vi "Measurement Logic.vi"(6 "NI GUID":string, 8 "error in":errorcluster, 9 "measurement configuration":T2 {"Baudrate" format="%x"; "FD Baudrate" format="%x"}, 10 "measure call context in":refnum<class "Measure Call Context.lvclass">, 11 "Stop OOB Server UE":refnum<user-event>) -> (0 "error out":errorcluster, 1 "measurement results":T1, 2 "measure call context out":refnum<class "Measure Call Context.lvclass">)   [LabVIEW 2025, in "CAN-LIN Raw Bus Capture.lvclass"]
doc: "Contains the core logic for executing the measurement."
uses:
  CAN-LIN Raw Bus Capture.lvclass
  <vilib>/Plug-In SDKs/Measurements/Measure Call Context/Measure Call Context.lvclass
  Measurement Configuration.ctl
  CAN-LIN Raw Bus Capture UI/Toggle.ctl
  Measurement Results.ctl
  Logic Data.ctl
  State.ctl
  Create Frame Buffer.vi
  <vilib>/xnet/xnet.llb/XNET Read (Frame LIN).vi
  <vilib>/xnet/xnet.llb/XNET Read (State LIN Comm).vi
  <vilib>/xnet/xnet.llb/XNET Read (Frame CAN).vi
  <vilib>/xnet/xnet.llb/XNET Read (State CAN Comm).vi
  Enqueue Frame.vi
  Destroy Frame Buffer.vi
  CAN-LIN Raw Bus Capture.lvclass/CAN-LIN Raw Bus Capture.ctl
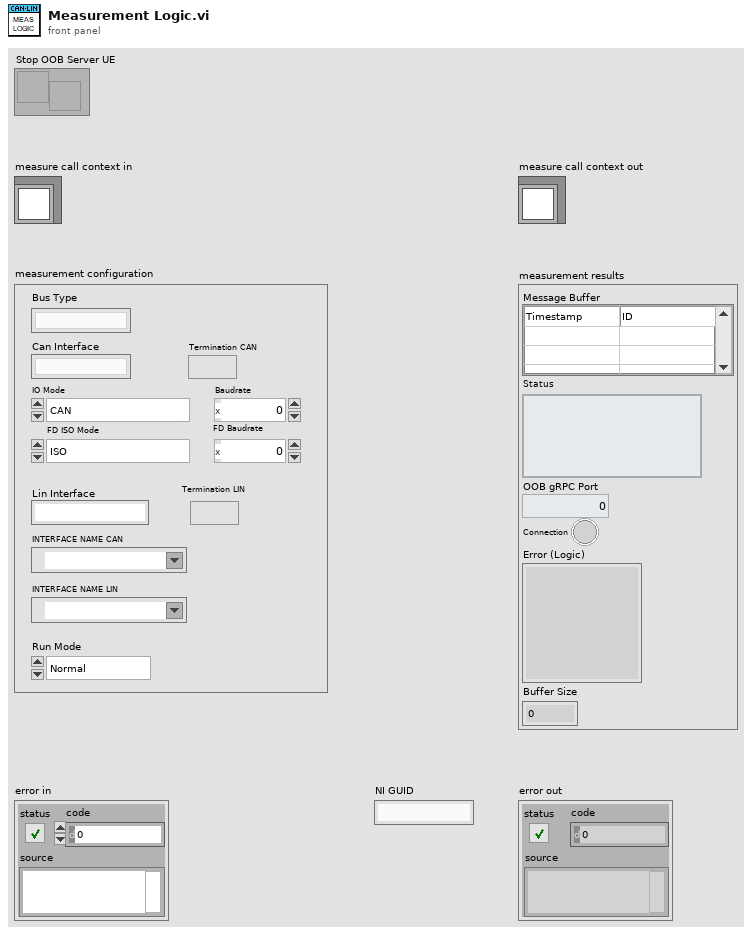
[diagram p1: front panel]
types:
  T1 = typedef "CAN-LIN Raw Bus Capture.lvclass/Measurement Results.ctl" = cluster{"Message Buffer":string[][], "Status":string, "OOB gRPC Port":i32, "Connection":bool, "Error (Logic)":string, "Buffer Size":i32}
  T2 = typedef "CAN-LIN Raw Bus Capture.lvclass/Measurement Configuration.ctl" = cluster{"Termination CAN":T3, "FD Baudrate":u32, "Baudrate":u32, "FD ISO Mode":enum32{"ISO", "Legacy ISO", "Non-ISO"}, "IO Mode":enum32{"CAN", "CAN FD", "CAN FD + BRS"}, "Termination LIN":T3, "Can Interface":string, "Lin Interface":string, "Bus Type":string, "INTERFACE NAME CAN":refnum<k21>, "INTERFACE NAME LIN":refnum<k21>, "Run Mode":enum32{"Normal", "Subordinate"}}
  T3 = typedef "Toggle.ctl" = bool
  T4 = typedef "CAN-LIN Raw Bus Capture.lvclass/Logic Data.ctl" = cluster{"State":T5, "Results":T1, "XNET Session":refnum<k21>}
  T5 = typedef "CAN-LIN Raw Bus Capture.lvclass/State.ctl" = enum16{"Init", "Execute", "Results", "Error", "Close"}
  T6 = typedef "XNET Frame LIN.ctl" = cluster{"timestamp":timestamp, "payload":u8[], "identifier":u32, "type":T7, "event ID":u8, "event slot?":bool, "echo?":bool}
  T7 = typedef "XNET Frame Type LIN.ctl" = u8
  T8 = typedef "XNET LIN Comm.ctl" = cluster{"fault code":i32, "fault?":bool, "communication state":T9, "last error":T10, "last error received":u8, "last error expected":u8, "last error identifier":u8, "sleep?":bool, "transceiver ready?":bool, "schedule index":u8}
  T9 = typedef "XNET LIN Comm State.ctl" = u8
  T10 = typedef "XNET LIN Last Err.ctl" = u8
  T11 = typedef "XNET Frame CAN.ctl" = cluster{"timestamp":timestamp, "payload":u8[], "identifier":u32, "type":T12, "extended?":bool, "echo?":bool}
  T12 = typedef "XNET Frame Type CAN.ctl" = u8
  T13 = typedef "XNET CAN Comm.ctl" = cluster{"fault code":i32, "fault?":bool, "communication state":T14, "last error":T15, "receive error counter":u8, "transmit error counter":u8, "transceiver error?":bool, "sleep?":bool}
  T14 = typedef "XNET CAN Comm State.ctl" = u8
  T15 = typedef "XNET CAN Last Err.ctl" = u8
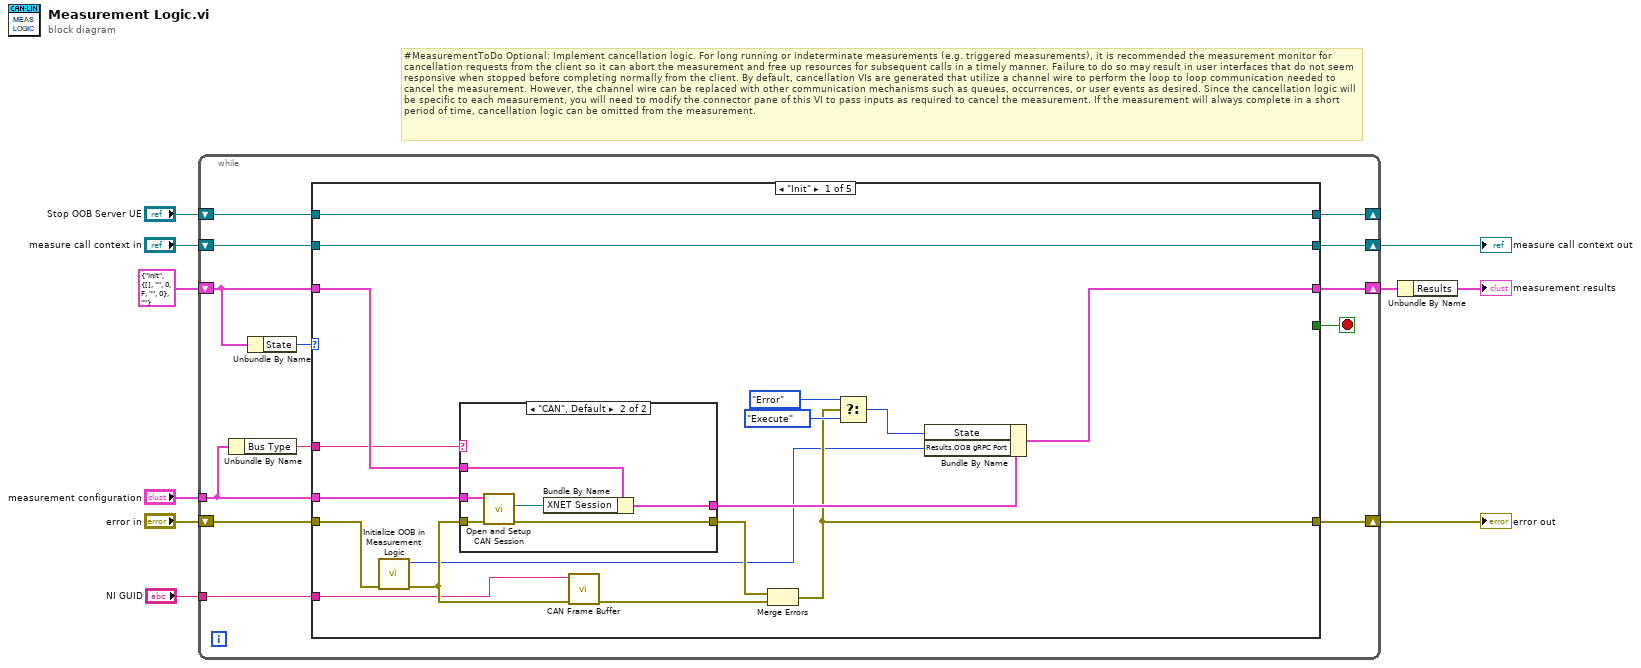
[diagram p0: block diagram]
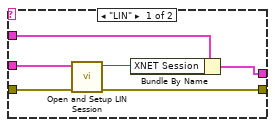
[diagram p2: hidden frame]
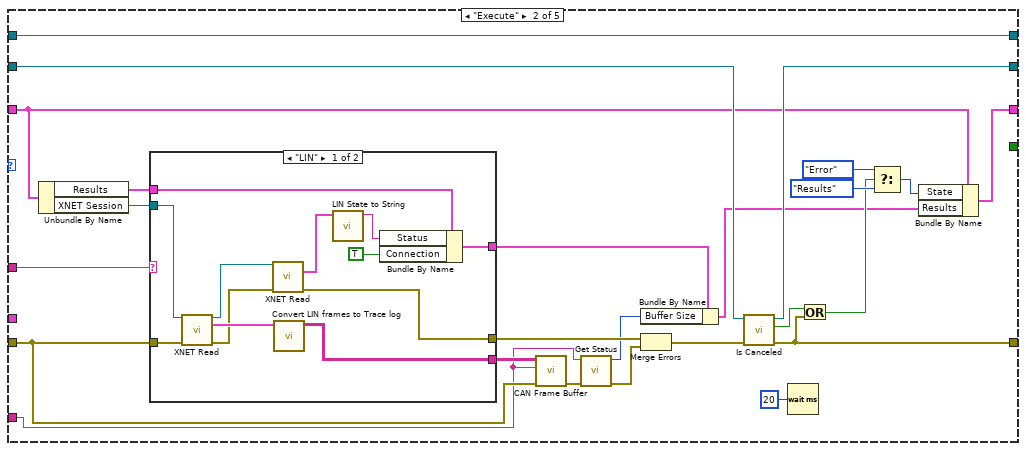
[diagram p3: hidden frame]
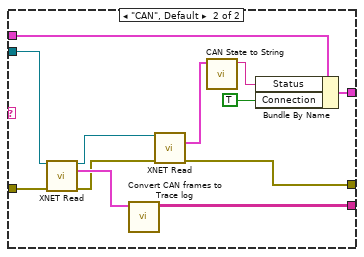
[diagram p4: hidden frame]
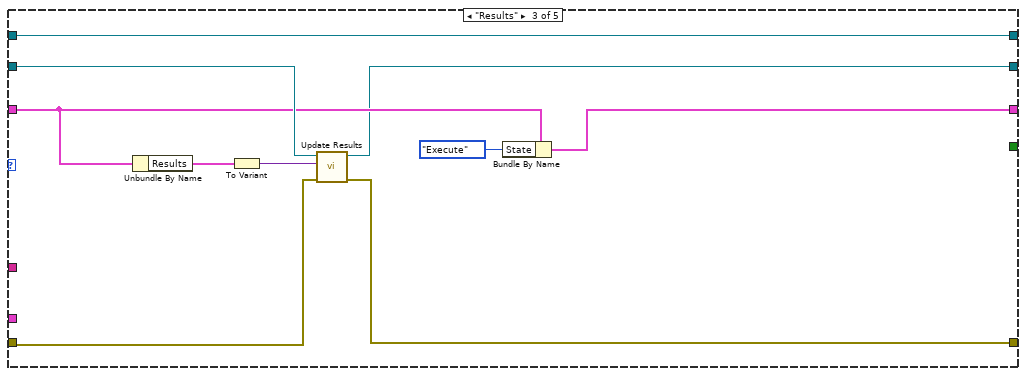
[diagram p5: hidden frame]
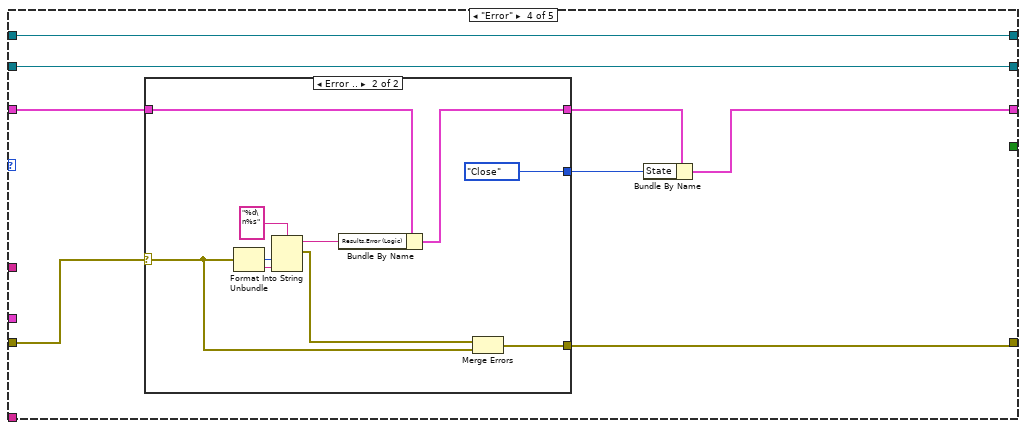
[diagram p6: hidden frame]
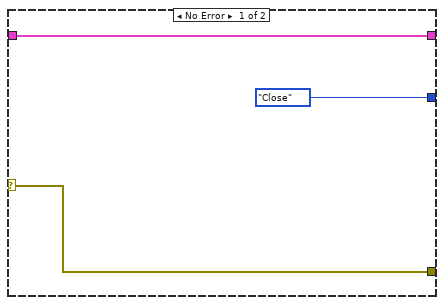
[diagram p7: hidden frame]
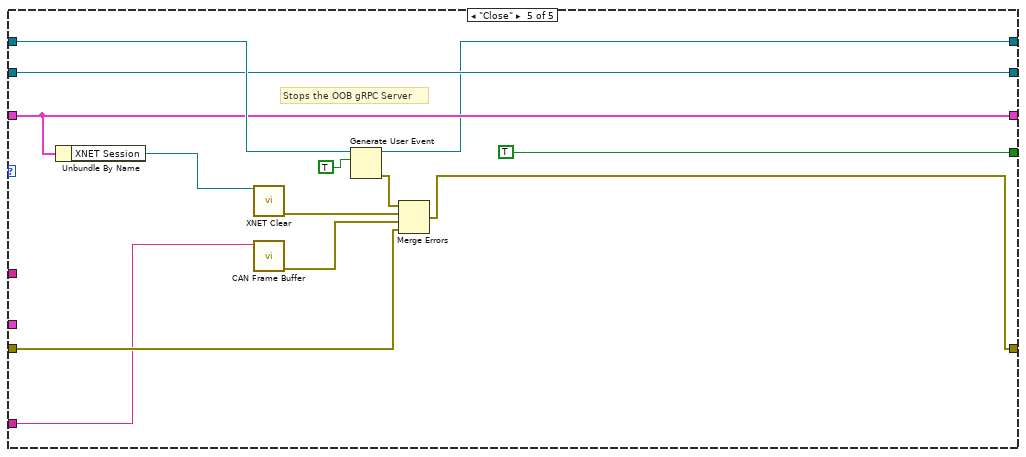
[diagram p8: hidden frame]
diagram:
  # "#MeasurementToDo Optional: Implement cancellation logic. For long running or indeterminate measurements (e.g. triggered measurements), it is recommended the measurement monitor for cancellation requests from the client so it can abort the measurement and free up resources for subsequent calls in a timely manner. Failure to do so may result in user interfaces that do not seem responsive when stopped before completing normally from the client. By default, cancellation VIs are generated that utilize a channel wire to perform the loop to loop communication needed to cancel the measurement. However, the channel wire can be replaced with other communication mechanisms such as queues, occurrences, or user events as desired. Since the cancellation logic will be specific to each measurement, you will need to modify the connector pane of this VI to pass inputs as required to cancel the measurement. If the measurement will always complete in a short period of time, cancellation logic can be omitted from the measurement."
  n1 = while {
    shift-right: [w19] -> w7
    shift-left: "error in" -> [w18]
    shift-right: [w20] -> w6
    shift-left: "measure call context in" -> [w23]
    shift-right: [w15] -> w3
    shift-left: T4 {"State"=enum."Init", "Results"={"Message Buffer"=[], "Status"="", "OOB gRPC Port"=0, "Connection"=FALSE, "Error (Logic)"="", "Buffer Size"=0}, "XNET Session"=""} ("Logic Data") -> [w16]
    tunnel: "measurement configuration" -> [w14]
    shift-right: [w12] -> _
    shift-left: "Stop OOB Server UE" -> [w22]
    tunnel: "NI GUID" -> [w11]
    stop <- w21 stop-if-true
    n2 = Unbundle By Name(w14) -> ("Bus Type"=w13:string)
    n3 = Unbundle By Name(w16) -> ("State"=w17:T5)
    n4 = case shown="\"Init\"" w17 {
      tunnel: w23 -> [w33 w73 w111 w113 w143]
      tunnel: w22 -> [w28 w57 w104 w112 w145]
      tunnel: [_ _ _ _ TRUE] -> w21
      tunnel: [w33 w69 w105 w113 w143] -> w20
      tunnel: [w32 w72 w109 w119 w144] -> w19
      tunnel: w18 -> [w26 w64 w110 w116 w136]
      tunnel: w16 -> [w34 w56 w108 w118 w138]
      tunnel: [w39 w59 w107 w115 w138] -> w15
      tunnel: w14 -> [w30 _ _ _ _]
      tunnel: w13 -> [w29 w60 _ _ _]
      tunnel: [w28 w57 w104 w112 w135] -> w12
      tunnel: w11 -> [w24 w53 _ _ w133]
      frame "Init" {
        n5 = call "Initialize OOB in Measurement Logic.vi"("error in"=w26) -> ("error out"=w27:errorcluster, "OBB Port"=w25:i32)  [unwired: 9 in]
        n6 = case shown="\"CAN\", Default" w29 {
          tunnel: [w45 w52] -> w40
          tunnel: [w42 w51] -> w35
          tunnel: w34 -> [w46 w50]
          tunnel: w30 -> [w43 w49]
          tunnel: w27 -> [w44 w47]
          frame "LIN" {
            n7 = call "Open and Setup LIN Session.vi"("error in"=w44, "measurement configuration"=w43) -> ("error out"=w42:errorcluster, "session out"=w41:refnum<k21>)  [unwired: 8 in]
            n8 = Bundle By Name(cluster=w46, "XNET Session"=w41) -> (w45:T4)
          }
          frame "CAN", Default {
            n9 = call "Open and Setup CAN Session.vi"("error in"=w47, "measurement configuration"=w49) -> ("error out"=w51:errorcluster, "session out"=w48:refnum<k21>)  [unwired: 8 in]
            n10 = Bundle By Name(cluster=w50, "XNET Session"=w48) -> (w52:T4)
          }
        }
        n11 = call-poly "CAN Frame Buffer.vi"("error in"=w27, "GUID"=w24) -> ("error out"=w31:errorcluster)  [unwired: 9 in]
        n12 = Merge Errors(w35, w31) -> (w32:errorcluster)
        n13 = Select(t=State."Error" ("State"), s=w32, f=State."Execute" ("State")) -> (s? t:f=w36:T5)
        n14 = Bundle By Name(cluster=w40, "State"=w36, "Results.OOB gRPC Port"=w25) -> (w39:T4)
      }
      frame "Execute" {
        n15 = Unbundle By Name(w56) -> ("Results"=w54:T1, "XNET Session"=w55:refnum<k21>)
        n16 = case shown="\"LIN\"" w60 {
          tunnel: w64 -> [w85 w101]
          tunnel: [w83 w96] -> w77
          tunnel: [w80 w95] -> w76
          tunnel: [w81 w92] -> w63
          tunnel: w55 -> [w79 w91]
          tunnel: w54 -> [w78 w90]
          frame "LIN" {
            n17 = call-poly <vilib>:"XNET Read.vi"("session in"=w79, "error in (no error)"=w85) -> ("session out"=w88:refnum<k21>, "data"=w89:T6[], "error out"=w86:errorcluster)  [unwired: 10 in, 1 out]
            n18 = call-poly <vilib>:"XNET Read.vi"("session in"=w88, "error in (no error)"=w86) -> ("LIN comm"=w87:T8, "error out"=w80:errorcluster)  [unwired: 11 in, 1 out]
            n19 = call "Convert LIN frames to Trace log.vi"("lin frames in"=w89) -> ("trace out"=w81:string[][])  [unwired: 10 in]
            n20 = call "LIN State to String.vi"("LIN comm in"=w87) -> ("string out"=w82:string)  [unwired: 10 in]
            n21 = Bundle By Name(cluster=w78, "Status"=w82, "Connection"=TRUE) -> (w83:T1)
          }
          frame "CAN", Default {
            n22 = call-poly <vilib>:"XNET Read.vi"("session in"=w91, "error in (no error)"=w101) -> ("session out"=w100:refnum<k21>, "data"=w94:T11[], "error out"=w93:errorcluster)  [unwired: 10 in, 1 out]
            n23 = call "Convert CAN frames to Trace log.vi"("can frames in"=w94) -> ("trace out"=w92:string[][])  [unwired: 10 in]
            n24 = call-poly <vilib>:"XNET Read.vi"("session in"=w100, "error in (no error)"=w93) -> ("CAN comm"=w99:T13, "error out"=w95:errorcluster)  [unwired: 11 in, 1 out]
            n25 = call "CAN State to String.vi"("CAN comm in"=w99) -> ("string out"=w98:string)  [unwired: 10 in]
            n26 = Bundle By Name(cluster=w90, "Status"=w98, "Connection"=TRUE) -> (w96:T1)
          }
        }
        n27 = call-poly "CAN Frame Buffer.vi"("error in"=w64, "GUID"=w53, "Data"=w63) -> ("error out"=w66:errorcluster)  [unwired: 7 in, 1 out]
        n28 = call "Get Status.vi"("error in"=w66, "GUID"=w53) -> ("error out"=w65:errorcluster, "Messages"=w61:i32)  [unwired: 8 in]
        n29 = Bundle By Name(cluster=w77, "Buffer Size"=w61) -> (w62:T1)
        n30 = Merge Errors(w76, w65) -> (w68:errorcluster)
        n31 = call <vilib>:"Is Canceled.vi"("error in"=w68, "measure call context in"=w73) -> ("error out"=w72:errorcluster, "is canceled?"=w71:bool, "measure call context out"=w69:refnum<class "Measure Call Context.lvclass">)  [unwired: 7 in]
        n32 = Wait (ms)(milliseconds to wait=u32 20) -> ()  [unwired: 1 out]
        n33 = Or(x=w71, y=w72) -> (x .or. y?=w70:bool)
        n34 = Select(t=State."Error" ("State"), s=w70, f=State."Results" ("State")) -> (s? t:f=w58:T5)
        n35 = Bundle By Name(cluster=w56, "State"=w58, "Results"=w62) -> (w59:T4)
      }
      frame "Results" {
        n36 = Unbundle By Name(w108) -> ("Results"=w103:T1)
        n37 = To Variant(anything=w103) -> (Variant=w102:variant)
        n38 = call <vilib>:"Update Results.vi"("error in"=w110, "measurement results"=w102, "measure call context in"=w111) -> ("error out"=w109:errorcluster, "measure call context out"=w105:refnum<class "Measure Call Context.lvclass">)  [unwired: 7 in]
        n39 = Bundle By Name(cluster=w108, "State"=State."Execute") -> (w107:T4)
      }
      frame "Error" {
        n40 = case shown="Error .." w116 {
          selector: w116 -> [w122 w123]
          tunnel: [w122 w124] -> w119
          tunnel: w118 -> [w120 w129]
          tunnel: [w120 w127] -> w117
          tunnel: [State."Close" ("State") State."Close" ("State")] -> w114
          frame No Error {
          }
          frame Error {
            n41 = Unbundle(w123) -> ("code"=w131:i32, "source"=w132:string)  [unwired: 1 out]
            n42 = Format Into String(format string="%d\n%s", w131, w132) -> (resulting string=w128:string, error out=w125:errorcluster)  [unwired: 2 in]
            n43 = Bundle By Name(cluster=w129, "Results.Error (Logic)"=w128) -> (w127:T4)
            n44 = Merge Errors(w125, w123) -> (w124:errorcluster)
          }
        }
        n45 = Bundle By Name(cluster=w117, "State"=w114) -> (w115:T4)
      }
      frame "Close" {
        # "Stops the OOB gRPC Server"
        n46 = Unbundle By Name(w138) -> ("XNET Session"=w137:refnum<k21>)
        n47 = call <vilib>:"XNET Clear.vi"("session in"=w137) -> ("error out"=w140:errorcluster)  [unwired: 14 in]
        n48 = call-poly "CAN Frame Buffer.vi"("GUID"=w133) -> ("error out"=w134:errorcluster)  [unwired: 10 in]
        n49 = Generate User Event(user event=w145, event data cluster=TRUE ("event data")) -> (user event out=w135:refnum<user-event>, error out=w141:errorcluster)  [unwired: 2 in]
        n50 = Merge Errors(w141, w140, w134, w136) -> (w144:errorcluster)
      }
    }
  }
  "error out" <- w7
  "measure call context out" <- w6
  n51 = Unbundle By Name(w3) -> ("Results"=→"measurement results":T1)
